vi "List-format.vi"(9 "RowHdrs[]":string[](array[string]), 10 "活动单元格:单元格大小":T1[](array[typedef])=[{"Width"=120, "Height"=50}, {"Width"=300, "Height"=50}, {"Width"=120, "Height"=50}], 11 "引用":refnum<vi>) -> ()   [LabVIEW 2018]
uses:
  <vilib>/Utility/miscctls.llb/LVBoundsTypeDef.ctl
  <vilib>/Utility/miscctls.llb/LVPositionTypeDef.ctl
panel:
  # "100行的多列列表字体大小更改\n+行首字符"
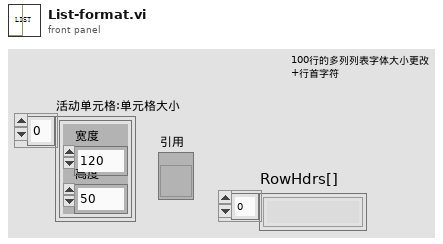
[diagram p1: front panel]
types:
  T1 = typedef "LVBoundsTypeDef.ctl" = cluster{"Width":u32, "Height":u32}
  T2 = typedef "LVPositionTypeDef.ctl" = cluster{"Left":i32, "Top":i32}
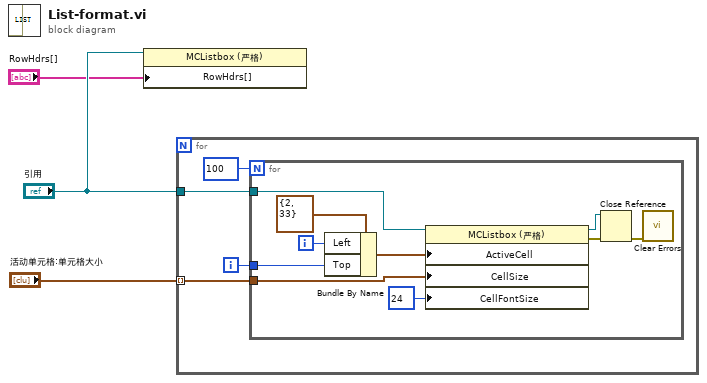
[diagram p0: block diagram]
diagram:
  n1 = property on="属性节点" class="MCListbox (严格)"(reference="引用", "RowHdrs[]"="RowHdrs[]") -> ()  [unwired: 1 in, 2 out]
  n2 = for {
    tunnel: "活动单元格:单元格大小" -> [w6] mode=indexing
    tunnel: "引用" -> [w4]
    i -> [w5]
    n3 = for {
      N: 100 -> [_]
      tunnel: w5 -> [w13]
      tunnel: w6 -> [w12]
      tunnel: w4 -> [w11]
      i -> [w14]
      n4 = Bundle By Name(cluster=T2 {"Left"=2, "Top"=33} ("活动单元格:位置"), "Left"=w14, "Top"=w13) -> (w15:T2)
      n5 = property on="属性节点" class="MCListbox (严格)"(reference=w11, "ActiveCell"=w15, "CellSize"=w12, "CellFontSize"=u32 24 ("活动单元格:单元格字体:字号")) -> (reference out=w10:refnum<vi>, error out=w9:errorcluster)  [unwired: 1 in]
      n6 = Close Reference(reference=w10, error in (no error)=w9) -> (error out=w8:errorcluster)
      n7 = call <vilib>:"Clear Errors.vi"("error in (no error)"=w8) -> ()  [unwired: 5 in, 2 out]
    }
  }
